vi "DDVL Adjust Spacing and Visibility.vi"(0 "Cluster Ref Array":refnum<vi>[](array[refnum]), 2 "Position Index":i32, 11 "Sub Panel Ref Array":refnum<vi>[](array[refnum]), 13 "Num of VIs":i32) -> (15 "Sub Panel Ref Array Dup":refnum<vi>[](array[refnum]))   [LabVIEW 2021]
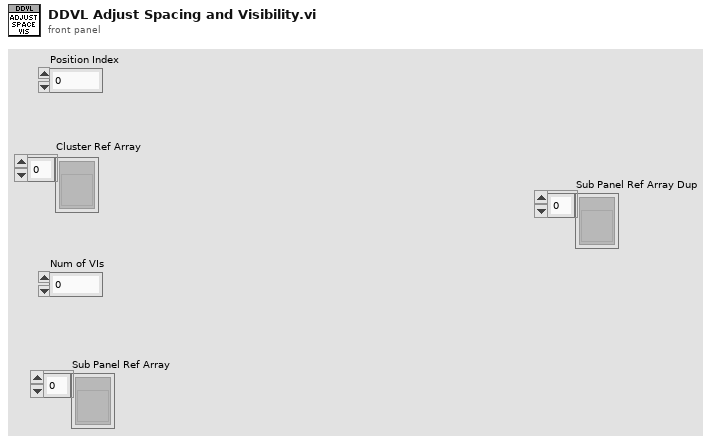
[diagram p1: front panel]
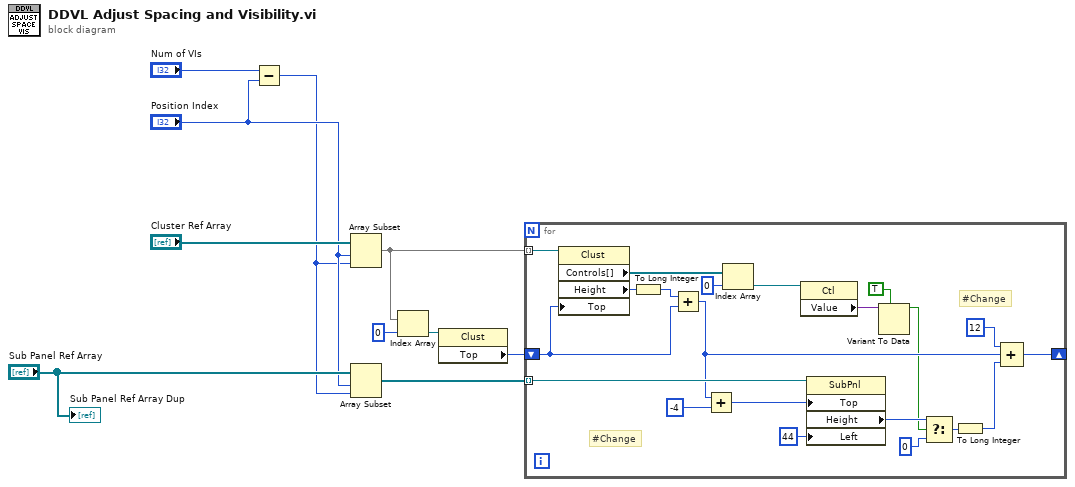
[diagram p0: block diagram]
diagram:
  n1 = Subtract(x="Num of VIs", y="Position Index") -> (x-y=w1:i32)
  n2 = Array Subset(array="Cluster Ref Array", index="Position Index", length=w1) -> (w7:refnum<vi>[])
  n3 = Array Subset(array="Sub Panel Ref Array", index="Position Index", length=w1) -> (w8:refnum<vi>[])
  n4 = Index Array(array=w7, index=0) -> (element=w5:refnum<vi>)
  n5 = property class="Clust"(reference=w5) -> ("Top"=w4:i32)  [unwired: 1 in, 2 out]
  n6 = for {
    tunnel: w7 -> [w31] mode=indexing
    tunnel: w8 -> [w28] mode=indexing
    shift-right: [w23] -> _
    shift-left: w4 -> [w20]
    # "#Change"
    # "#Change"
    n7 = property class="Clust"(reference=w31, "Top"=w20) -> ("Controls[]"=w18:refnum<vi>[], "Height"=w30:u32)  [unwired: 1 in, 2 out]
    n8 = To Long Integer(number=w30) -> (32bit integer=w29:i32)
    n9 = Add(x=w29, y=w20) -> (x+y=w19:i32)
    n10 = Add(x=w19, y=-4 ("Offset Adjust")) -> (x+y=w11:i32)
    n11 = Index Array(array=w18, index=0) -> (element=w16:refnum<vi>)
    n12 = property class="Ctl"(reference=w16) -> ("Value"=w15:variant)  [unwired: 1 in, 2 out]
    n13 = property class="SubPnl"(reference=w28, "Top"=w11, "Left"=44 ("Position:Left")) -> ("Height"=w26:u32)  [unwired: 1 in, 2 out]
    n14 = Variant To Data(type=TRUE, Variant=w15) -> (data=w13:bool)  [unwired: 1 in, 1 out]
    n15 = Select(t=w26, s=w13, f=u32 0) -> (s? t:f=w24:u32)
    n16 = To Long Integer(number=w24) -> (32bit integer=w21:i32)
    n17 = Compound Arithmetic op=ADD(12 ("x"), w19, w21) -> (w23:i32)
  }
  "Sub Panel Ref Array Dup" <- "Sub Panel Ref Array"
